vi "SPARK Get Alt Ext Encoder Config.vi"   [LabVIEW 2027]
doc: "Get the configuration of the alternate or external encoder connected to the data port of the SPARK."
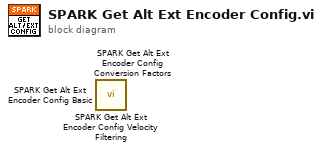
[diagram p0: block diagram]
diagram:
  n1 = call <vilib>:"SPARK Get Alt Ext Encoder Config Velocity Filtering.vi"() -> ()  [unwired: 8 in, 4 out]
  n2 = call <vilib>:"SPARK Get Alt Ext Encoder Config Conversion Factors.vi"() -> ()  [unwired: 8 in, 4 out]
  n3 = call <vilib>:"SPARK Get Alt Ext Encoder Config Basic.vi"() -> ()  [unwired: 8 in, 4 out]
